vi "SetWindowLongPtrW Wrapper Template.vi"(0 "hWnd":u64, 5 "nIndex":i32=-20, 7 "dwNewLong":i64, 11 "error in":errorcluster) -> (4 "return value":i64, 15 "error out":errorcluster)   [LabVIEW 2020]
doc: "Writes a value of the window hWnd through user32.dll SetWindowLongPtrW (stdcall, called in any thread). nIndex -16 GWL_STYLE sets the window style, -20 GWL_EXSTYLE the extended style (WS_EX_LAYERED 0x80000). return value is the previous value; 0 can mean failure. When error in carries an error the DLL is not called. Generated by tools\\Build Win32 Wrappers.vi - do not edit by hand, rebuild it."
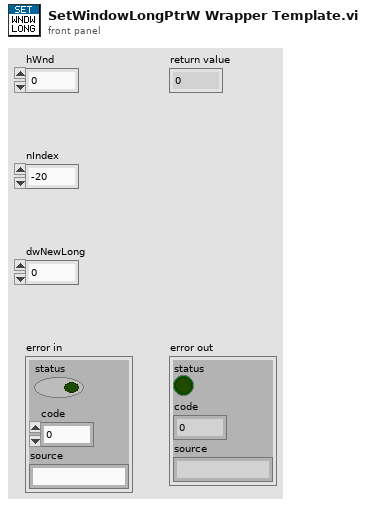
[diagram p1: front panel]
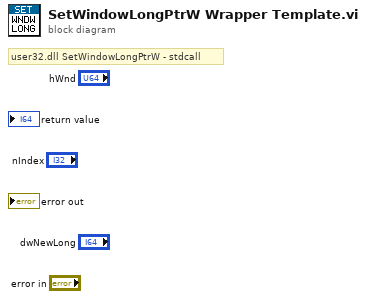
[diagram p0: block diagram]
diagram:
  # "user32.dll SetWindowLongPtrW - stdcall"
